vi "VIH Utility - STR - Filter 1D Array of Strings (w patterns).vi"(8 "Action (keep instances)":enum16{"keep instances", "remove instances"}(ring), 10 "Regular expressions":string[](array[string]), 11 "Array in":string[](array[string])) -> (3 "Array out":string[](array[string]))   [LabVIEW 2014]
doc: "::: VI Helpeks :::\nCopyright (c) 2000-2026 Konstantin Shifershteyn. All rights reserved."
panel:
  # "VI Helpeks\nCopyright (c) 2012-2026 Konstantin Shifershteyn"
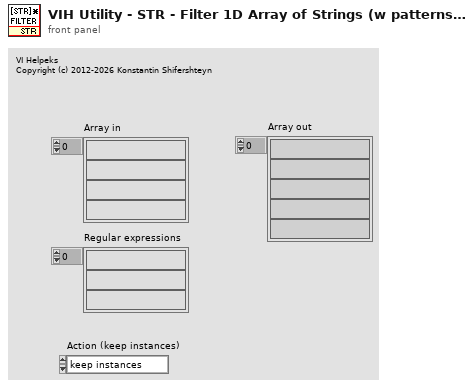
[diagram p1: front panel]
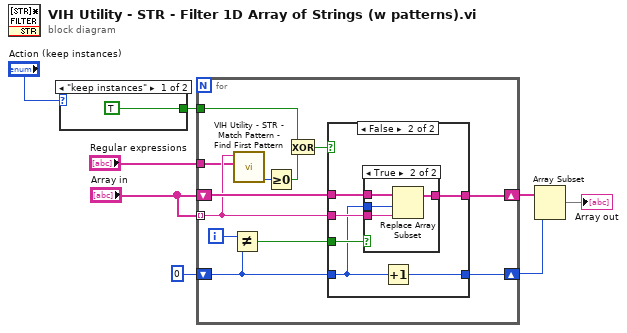
[diagram p0: block diagram]
diagram:
  n1 = case shown="\"keep instances\"" "Action (keep instances)" {
    tunnel: [TRUE _] -> w3
    frame "keep instances" {
    }
    frame "remove instances" {
    }
  }
  n2 = for {
    tunnel: "Regular expressions" -> [w11]
    shift-right: [w19] -> w8
    shift-left: "Array in" -> [w21]
    tunnel: "Array in" -> [w12] mode=indexing
    shift-right: [w20] -> w1
    shift-left: 0 -> [w16]
    tunnel: w3 -> [w14]
    i -> [w17]
    n3 = Not Equal?(x=w17, y=w16) -> (x != y?=w18:bool)
    n4 = call "VIH Utility - STR - Match Pattern - Find First Pattern.vi"("Regular expressions"=w11, "String"=w12) -> ("offset past match"=w10:i32)  [unwired: 2 in, 5 out]
    n5 = Greater Or Equal To 0?(x=w10) -> (x >= 0?=w15:bool)
    n6 = Exclusive Or(1:w15, 2:w14) -> (0:w13:bool)
    n7 = case shown="False" w13 {
      tunnel: w21 -> [w23 w29]
      tunnel: w12 -> [_ w28]
      tunnel: w16 -> [w22 w25]
      tunnel: [w22 w24] -> w20
      tunnel: [w23 w27] -> w19
      tunnel: w18 -> [_ w26]
      frame True {
      }
      frame False {
        n8 = case shown="True" w26 {
          tunnel: w29 -> [w30 w34]
          tunnel: w28 -> [_ w33]
          tunnel: [w30 w32] -> w27
          tunnel: w25 -> [_ w31]
          frame False {
          }
          frame True {
            n9 = Replace Array Subset(array=w34, new element=w33, index=w31) -> (w32:string[])
          }
        }
        n10 = Increment(x=w25) -> (x+1=w24:i32)
      }
    }
  }
  n11 = Array Subset(array=w8, length=w1) -> (→"Array out":string[])  [unwired: 1 in]
